vi "JUnit Full.vi"() -> ()   [LabVIEW 2013]
doc: "This example illustrates how to create a complete JUnit XML report."
uses:
  JUnit XML/Test Suites/Test Suites.lvclass
  JUnit XML/Test Case/Test Case.lvclass
  JUnit XML/Test Suite/Test Suite.lvclass
  JUnit XML/Property/Property.lvclass
panel:
  out "XML":string
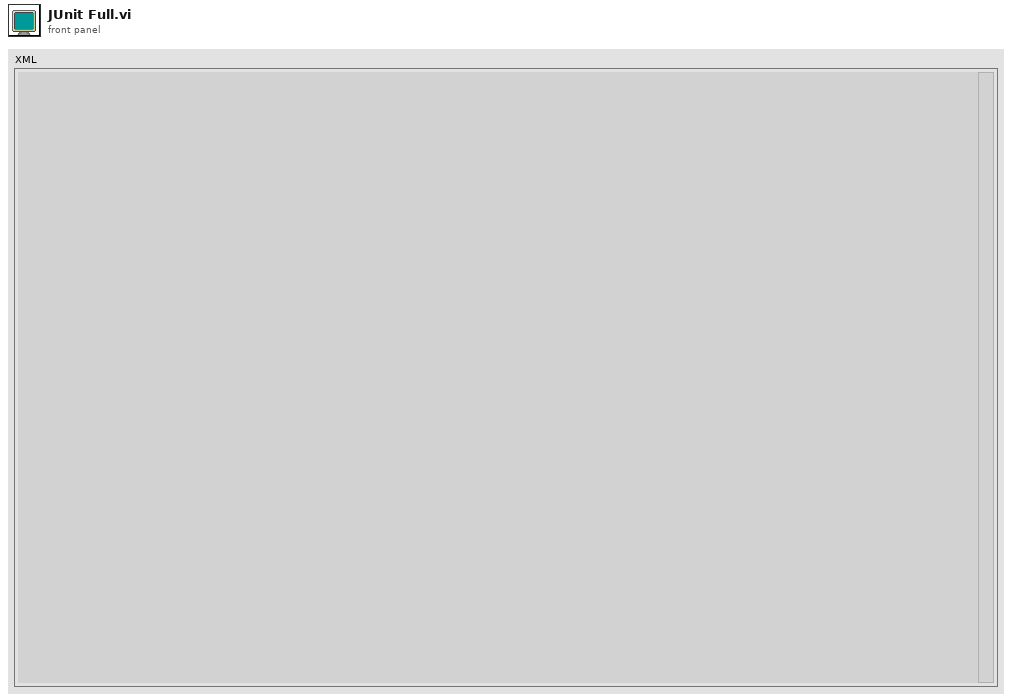
[diagram p1: front panel]
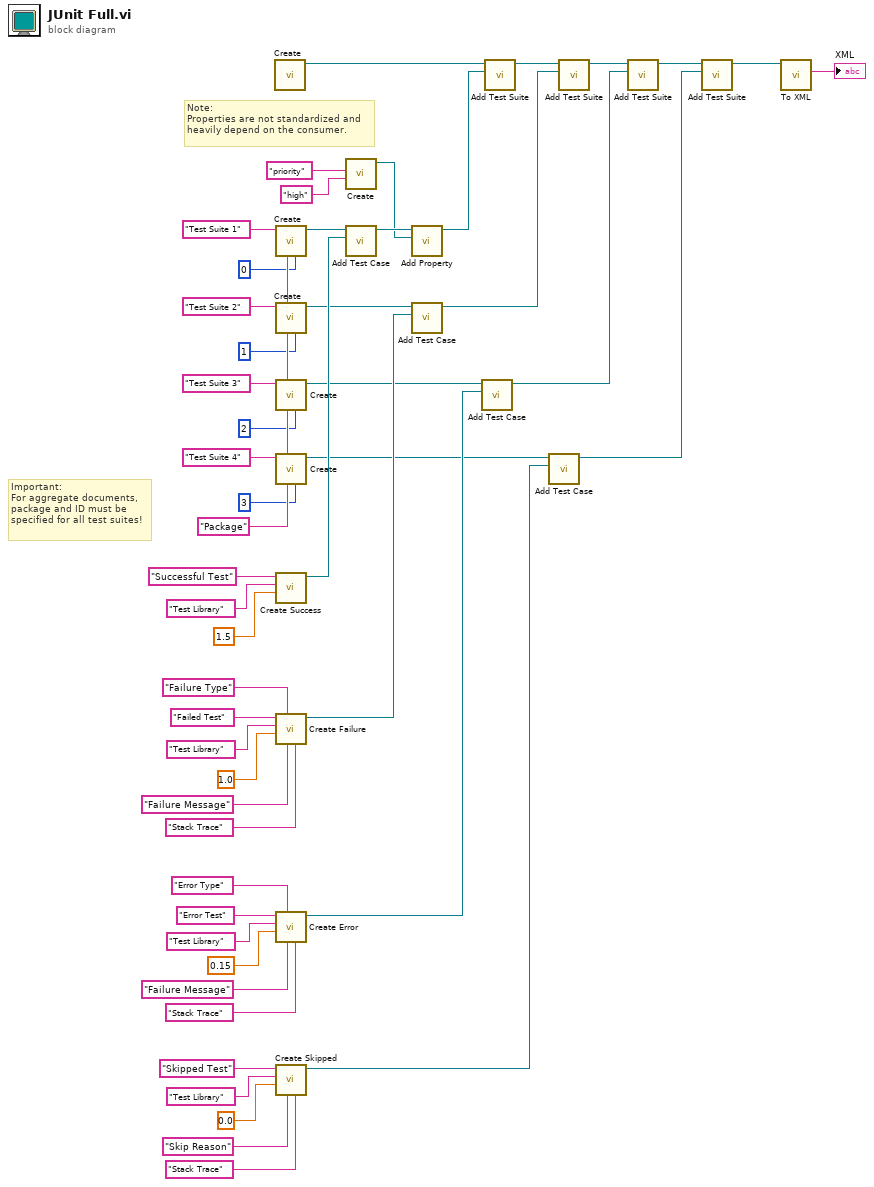
[diagram p0: block diagram]
diagram:
  w11 = "Package" ("Package (\"\" = undefined)")
  # "Note:\nProperties are not standardized and\nheavily depend on the consumer."
  # "Important:\nFor aggregate documents,\npackage and ID must be\nspecified for all test suites!"
  n1 = call "Create.vi"() -> ("Test Suites"=w25:refnum<class "Test Suites.lvclass">)  [unwired: 10 in, 1 out]
  n2 = call "Create.vi"("Id (-1 = undefined)"=0, "Package (\"\" = undefined)"=w11, "Name"="Test Suite 1") -> ("Test Suite"=w47:refnum<class "Test Suite.lvclass">)  [unwired: 7 in, 1 out]
  n3 = call "Create.vi"("Id (-1 = undefined)"=1, "Package (\"\" = undefined)"=w11, "Name"="Test Suite 2") -> ("Test Suite"=w21:refnum<class "Test Suite.lvclass">)  [unwired: 7 in, 1 out]
  n4 = call "Create.vi"("Id (-1 = undefined)"=2, "Package (\"\" = undefined)"=w11, "Name"="Test Suite 3") -> ("Test Suite"=w20:refnum<class "Test Suite.lvclass">)  [unwired: 7 in, 1 out]
  n5 = call "Create.vi"("Id (-1 = undefined)"=3, "Package (\"\" = undefined)"=w11, "Name"="Test Suite 4") -> ("Test Suite"=w19:refnum<class "Test Suite.lvclass">)  [unwired: 7 in, 1 out]
  n6 = call "Create Success.vi"("Time"=1.5, "Classname"="Test Library", "Name"="Successful Test") -> ("Test Case"=w46:refnum<class "Test Case.lvclass">)  [unwired: 7 in, 1 out]
  n7 = call "Create Failure.vi"("Stack Trace"="Stack Trace", "Message"="Failure Message", "Type"="Failure Type", "Time"=1.0, "Classname"="Test Library", "Name"="Failed Test") -> ("Test Case"=w39:refnum<class "Test Case.lvclass">)  [unwired: 4 in, 1 out]
  n8 = call "Create Error.vi"("Stack Trace"="Stack Trace", "Message"="Failure Message", "Type"="Error Type", "Time"=0.15, "Classname"="Test Library", "Name"="Error Test") -> ("Test Case"=w32:refnum<class "Test Case.lvclass">)  [unwired: 4 in, 1 out]
  n9 = call "Create Skipped.vi"("Stack Trace"="Stack Trace", "Message"="Skip Reason", "Time"=0.0, "Classname"="Test Library", "Name"="Skipped Test") -> ("Test Case"=w26:refnum<class "Test Case.lvclass">)  [unwired: 5 in, 1 out]
  n10 = call "Create.vi"("Value"="high", "Name"="priority") -> ("Property"=w4:refnum<class "Property.lvclass">)  [unwired: 8 in, 1 out]
  n11 = call "Add Test Case.vi"("Test Case"=w46, "Test Suite in"=w47) -> ("Test Suite out"=w6:refnum<class "Test Suite.lvclass">)  [unwired: 8 in, 1 out]
  n12 = call "Add Property.vi"("Property"=w4, "Test Suite in"=w6) -> ("Test Suite out"=w5:refnum<class "Test Suite.lvclass">)  [unwired: 8 in, 1 out]
  n13 = call "Add Test Case.vi"("Test Case"=w39, "Test Suite in"=w21) -> ("Test Suite out"=w17:refnum<class "Test Suite.lvclass">)  [unwired: 8 in, 1 out]
  n14 = call "Add Test Case.vi"("Test Case"=w32, "Test Suite in"=w20) -> ("Test Suite out"=w16:refnum<class "Test Suite.lvclass">)  [unwired: 8 in, 1 out]
  n15 = call "Add Test Suite.vi"("Test Suite"=w5, "Test Suites in"=w25) -> ("Test Suites out"=w18:refnum<class "Test Suites.lvclass">)  [unwired: 8 in, 1 out]
  n16 = call "Add Test Case.vi"("Test Case"=w26, "Test Suite in"=w19) -> ("Test Suite out"=w14:refnum<class "Test Suite.lvclass">)  [unwired: 8 in, 1 out]
  n17 = call "Add Test Suite.vi"("Test Suite"=w17, "Test Suites in"=w18) -> ("Test Suites out"=w15:refnum<class "Test Suites.lvclass">)  [unwired: 8 in, 1 out]
  n18 = call "Add Test Suite.vi"("Test Suite"=w16, "Test Suites in"=w15) -> ("Test Suites out"=w13:refnum<class "Test Suites.lvclass">)  [unwired: 8 in, 1 out]
  n19 = call "Add Test Suite.vi"("Test Suite"=w14, "Test Suites in"=w13) -> ("Test Suites out"=w12:refnum<class "Test Suites.lvclass">)  [unwired: 8 in, 1 out]
  n20 = call-dynamic "To XML.vi"("Serializable in"=w12) -> ("XML"=→"XML":string)  [unwired: 9 in, 1 out]
